vi "Arreglo_Bidimensional.vi"() -> ()   [LabVIEW 2026]
panel:
  out "INDICADOR":dbl[][](array[numeric])
  in  "NUEVO VALOR":dbl
  in  "COLUMNA":i16
  in  "FILA":i16
  in  "ORIGINAL":dbl[][](array[numeric])
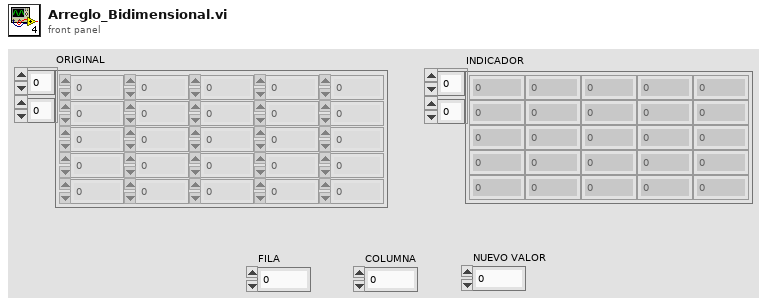
[diagram p1: front panel]
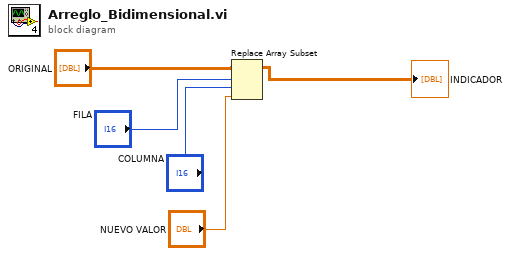
[diagram p0: block diagram]
diagram:
  n1 = Replace Array Subset(array="ORIGINAL", new element="NUEVO VALOR", index (row)="FILA", index (col)="COLUMNA") -> (→"INDICADOR":dbl[][])
